vi "get dataset by rid.vi"(10 "Dataset RID":string, 11 "connection":refnum<class "Nominal Client.lvclass">) -> (0 "error out":errorcluster, 3 "Dataset":refnum<class "dataset.lvclass">)   [LabVIEW 2020, in "nominal core steps.lvlib"]
doc: "Using a dataset RID, get a reference to the dataset object. This can then be used to create a Stream.\n<b> </b> <b> </b>"
uses:
  nominal core steps.lvlib
  <vilib>/Nominal/Nominal IO Client/lv_src/Nominal Client/Nominal Client.lvclass
  <vilib>/Nominal/Nominal IO Client/lv_src/datasources/dataset/dataset.lvclass
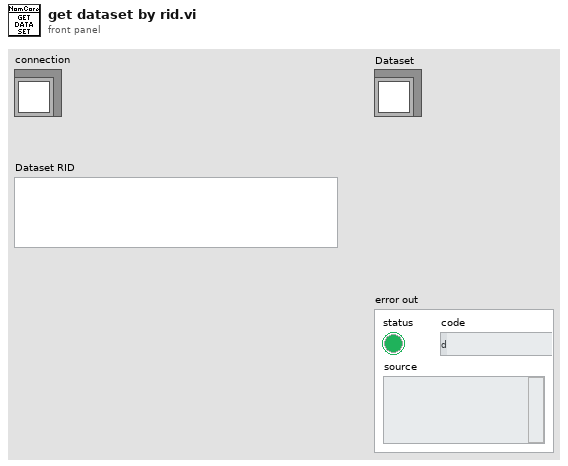
[diagram p1: front panel]
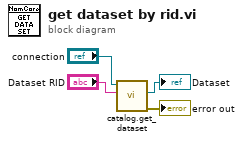
[diagram p0: block diagram]
diagram:
  n1 = call <vilib>:"catalog.get_dataset.vi"("Dataset RID"="Dataset RID", "Nominal Client in"="connection") -> ("error out"=→"error out":errorcluster, "Dataset"=→"Dataset":refnum<class "dataset.lvclass">)  [unwired: 7 in, 1 out]
